vi "tSNIP_power_level_analog_output.vi"(8 "Safely stop":bool, 9 "DAQmx Device Name":tag, 10 "LASER ON":bool, 11 "LASER power (mW)":dbl min=0.0 max=5000.0 step=20.0) -> ()   [LabVIEW 2025]
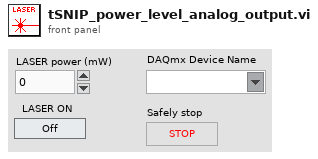
[diagram p1: front panel]
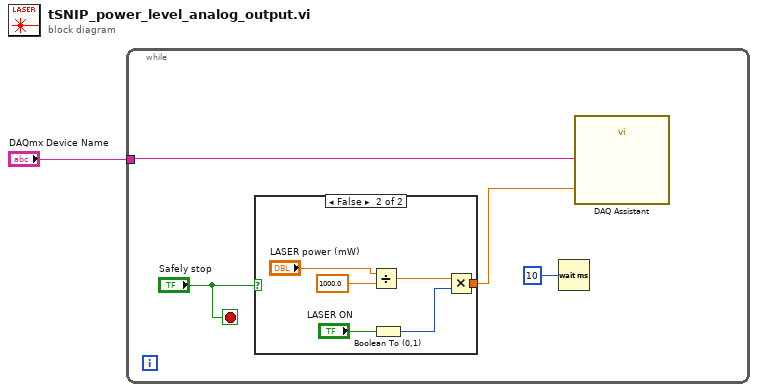
[diagram p0: block diagram]
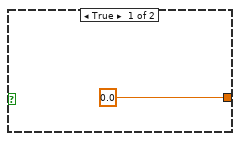
[diagram p2: hidden frame]
diagram:
  n1 = while {
    tunnel: "DAQmx Device Name" -> [w5]
    stop <- "Safely stop" stop-if-true
    n2 = case shown="False" "Safely stop" {
      tunnel: [0.0 w7] -> w4
      frame True {
      }
      frame False {
        n3 = Divide(x="LASER power (mW)", y=1000.0) -> (x/y=w11:dbl)
        n4 = Boolean To (0,1)(Boolean="LASER ON") -> (0, 1=w12:i16)
        n5 = Multiply(x=w11, y=w12) -> (x*y=w7:dbl)
      }
    }
    n6 = Wait (ms)(milliseconds to wait=u32 10) -> ()  [unwired: 1 out]
    n7 = call "DAQ Assistant"("data"=w4, "device name"=w5) -> ()  [unwired: 16 in, 2 out]
  }
